vi "Sous_VI_Virage_Gauche.vi"(8 "error in (no error)":errorcluster, 9 "Angle rotation degres":i32, 11 "Choix rotation":T1) -> (0 "error out":errorcluster)   [LabVIEW 2017]
uses:
  enum_rotation_robot.ctl
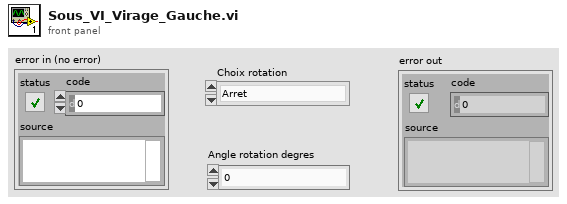
[diagram p1: front panel]
types:
  T1 = typedef "enum_rotation_robot.ctl" = enum16{"Arret", "Rotation_gauche", "Rotation_droite"}
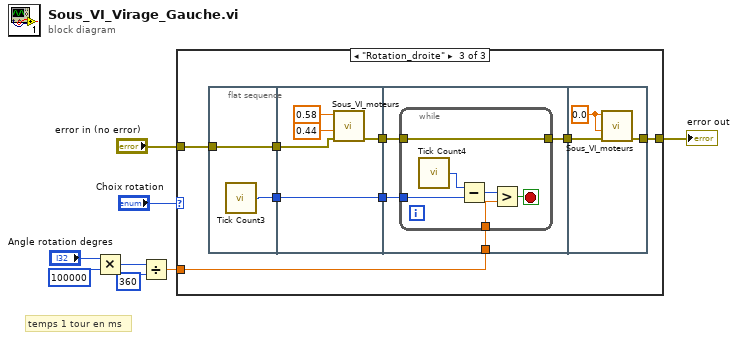
[diagram p0: block diagram]
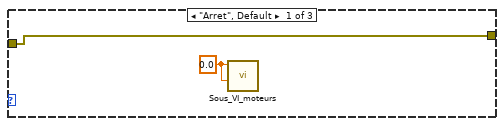
[diagram p2: hidden frame]
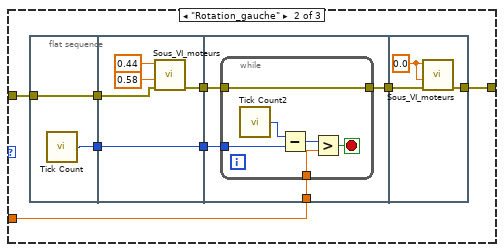
[diagram p3: hidden frame]
diagram:
  # "temps 1 tour en ms"
  n1 = Multiply(x="Angle rotation degres", y=100000) -> (x*y=w7:i32)
  n2 = Divide(x=w7, y=360) -> (x/y=w3:dbl)
  n3 = case shown="\"Rotation_droite\"" "Choix rotation" {
    tunnel: w3 -> [_ w16 w41]
    tunnel: "error in (no error)" -> [w9 w13 w40]
    tunnel: [w9 w11 w39] -> w1
    frame "Arret", Default {
      w10 = 0.0 ("Moteur Gauche")
      n4 = call "Sous_VI_moteurs.vi"("Moteur Droit"=w10, "Moteur Gauche"=w10) -> ()  [unwired: 9 in, 1 out]
    }
    frame "Rotation_gauche" {
      n5 = flat-sequence {
        tunnel: [w20] -> w17
        tunnel: w13 -> [w19]
        tunnel: [w19] -> w12
        tunnel: [w24] -> w18
        tunnel: w17 -> [w24]
        tunnel: [w22] -> w15
        tunnel: w12 -> [w21]
        tunnel: w18 -> [w29]
        tunnel: w16 -> [w28]
        tunnel: w15 -> [w27]
        tunnel: [w26] -> w14
        tunnel: w14 -> [w37]
        tunnel: [w36] -> w11
        frame #0 {
          n6 = call "Tick Count"() -> ("Tick Count(mSec)"=w20:u32)
        }
        frame #1 {
          n7 = call "Sous_VI_moteurs.vi"("error in (no error)"=w21, "Moteur Droit"=0.58, "Moteur Gauche"=0.44) -> ("error out"=w22:errorcluster)  [unwired: 8 in]
        }
        frame #2 {
          n8 = while {
            tunnel: w29 -> [w34]
            tunnel: w28 -> [w32]
            tunnel: w27 -> [w30]
            tunnel: [w30] -> w26
            stop <- w31 stop-if-true
            n9 = call "Tick Count2"() -> ("Tick Count(mSec)"=w35:u32)
            n10 = Subtract(x=w35, y=w34) -> (x-y=w33:u32)
            n11 = Greater?(x=w33, y=w32) -> (0:w31:bool)
          }
        }
        frame #3 {
          w38 = 0.0 ("Moteur Gauche")
          n12 = call "Sous_VI_moteurs.vi"("error in (no error)"=w37, "Moteur Droit"=w38, "Moteur Gauche"=w38) -> ("error out"=w36:errorcluster)  [unwired: 8 in]
        }
      }
    }
    frame "Rotation_droite" {
      n13 = flat-sequence {
        tunnel: [w48] -> w46
        tunnel: w40 -> [w47]
        tunnel: [w47] -> w45
        tunnel: [w52] -> w44
        tunnel: w46 -> [w52]
        tunnel: [w50] -> w43
        tunnel: w45 -> [w49]
        tunnel: w44 -> [w57]
        tunnel: w41 -> [w56]
        tunnel: w43 -> [w55]
        tunnel: [w54] -> w42
        tunnel: w42 -> [w65]
        tunnel: [w64] -> w39
        frame #0 {
          n14 = call "Tick Count3"() -> ("Tick Count(mSec)"=w48:u32)
        }
        frame #1 {
          n15 = call "Sous_VI_moteurs.vi"("error in (no error)"=w49, "Moteur Droit"=0.44, "Moteur Gauche"=0.58) -> ("error out"=w50:errorcluster)  [unwired: 8 in]
        }
        frame #2 {
          n16 = while {
            tunnel: w57 -> [w62]
            tunnel: w56 -> [w60]
            tunnel: w55 -> [w58]
            tunnel: [w58] -> w54
            stop <- w59 stop-if-true
            n17 = call "Tick Count4"() -> ("Tick Count(mSec)"=w63:u32)
            n18 = Subtract(x=w63, y=w62) -> (x-y=w61:u32)
            n19 = Greater?(x=w61, y=w60) -> (0:w59:bool)
          }
        }
        frame #3 {
          w66 = 0.0 ("Moteur Gauche")
          n20 = call "Sous_VI_moteurs.vi"("error in (no error)"=w65, "Moteur Droit"=w66, "Moteur Gauche"=w66) -> ("error out"=w64:errorcluster)  [unwired: 8 in]
        }
      }
    }
  }
  "error out" <- w1
